vi "Basic Function Generator (Absolute Time).vi"(3 "offset":dbl format="%0.2p", 4 "square wave duty cycle (%)":dbl=50.0 format="%0.2f", 5 "reset signal":bool, 6 "sampling info":cluster{"Fs":dbl, "#s":dbl}={"Fs"=1000.0, "#s"=1000.0} {"Fs" format="%.2p"}, 7 "signal type":T1(ring), 8 "error in (no error)":errorcluster, 9 "phase":dbl format="%.2p", 10 "amplitude":dbl=1.0 format="%0.2p", 11 "frequency":dbl=10.0 format="%0.2p") -> (0 "error out":errorcluster, 1 "phase out":dbl format="%.2p", 2 "signal out":waveform(dbl))   [LabVIEW 2020, in "Nominal Streaming.lvlib"]
uses:
  Channel.lvclass/Channel.ctl
  Nominal Streaming/Nominal Streaming.lvlib
  <vilib>/measure/NI_MABase.lvlib
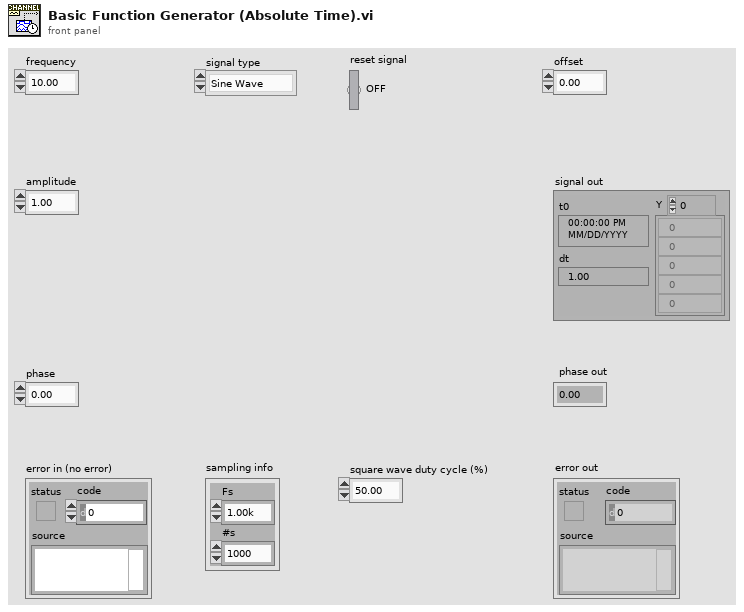
[diagram p1: front panel]
types:
  T1 = enum16{"Sine Wave", "Triangle Wave", "Square Wave", "Sawtooth Wave"}
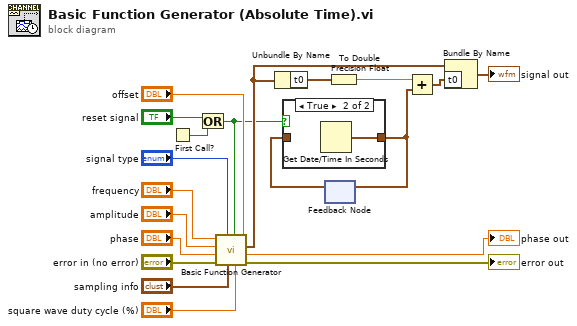
[diagram p0: block diagram]
diagram:
  n1 = First Call?() -> (First Call?: T/F=w5:bool)
  n2 = Or(x="reset signal", y=w5) -> (x .or. y?=w3:bool)
  n3 = call <vilib>:"Basic Function Generator.vi"("offset"="offset", "square wave duty cycle (%)"="square wave duty cycle (%)", "reset signal"=w3, "sampling info"="sampling info", "signal type"="signal type", "error in (no error)"="error in (no error)", "phase"="phase", "amplitude"="amplitude", "frequency"="frequency") -> ("error out"=→"error out":errorcluster, "phase out"=→"phase out":dbl, "signal out"=w20:waveform(dbl))
  n4 = Unbundle By Name(w20) -> ("t0"=w19:timestamp)
  n5 = feedback #1() -> (w1:timestamp)  [unwired: 1 in]
  n6 = case shown="True" w3 {
    tunnel: [w21 w22] -> w2
    tunnel: w1 -> [w21 _]
    frame False {
    }
    frame True {
      n7 = Get Date/Time In Seconds() -> (seconds since 1Jan1904=w22:timestamp)
    }
  }
  n8 = feedback-in #1(w2) -> ()
  n9 = To Double Precision Float(number=w19) -> (double precision float=w18:dbl)
  n10 = Add(x=w18, y=w2) -> (x+y=w17:timestamp)
  n11 = Bundle By Name(cluster=w20, "t0"=w17) -> (→"signal out":waveform(dbl))
